vi "Machine Setting - Read Write Machine (SubVI).vi"() -> ()   [LabVIEW 2019]
uses:
  Controls/MachineSetting-state.ctl
  Controls/UDP - Command.ctl
  Controls/Communication - Write Data.ctl
  <vilib>/Utility/sysdir.llb/System Directory Type.ctl
  Controls/Global - Data UDP.vi
  <vilib>/Utility/config.llb/Write Key (String).vi
  <vilib>/Utility/config.llb/Read Key (String).vi
  <vilib>/Utility/config.llb/NI_LVConfig.lvlib
panel:
  in  "Save":bool
  in  "Load":bool
  in  "IP Address":string
  in  "Set":bool
  in  "Get":bool
  in  "Tab Control":enum32{"System", "Test", "ADC", "Sensor", "PID"}(tab)
  in  "System":string[][](table)=[["Out_Type"], ["Inverse"], ["Monitor"], ["ACC_Time"], ["Pulse_rev"], ["Stroke"], ["Auto Off"], ["Gear_Ratio"], ["Pitch"], ["Max Speed"], ["Jog Speed"], ["Disp Coff"], ["Max Load"]]
  in  "Test":string[][](table)=[["Traget #1"], ["Target #2"], ["Speed #1"], ["Speed #2"], [""], [""], [""], [""], [""], [""], [""], [""]]
  in  "ADC":string[][](table)=[["ActiveCH #0"], ["ActiveCH #1"], ["ActiveCH #2"], ["ActiveCH #3"], ["ActiveCH #4"], ["ActiveCH #5"], ["ActiveCH #6"], ["ActiveCH #7"], ["FilterType"], ["PostFilter #0"], ["PostFilter #1"], ["PostFilter #2"], ["PostFilter #3"], ["PostFilter #4"], ["PostFilter #5"], ["PostFilter #6"], ["PostFilter #7"], ["Gain #0"], ["Gain #1"], ["Gain #2"], ["Gain #3"], ["Gain #4"], ["Gain #5"], ["Gain #6"], ["Gain #7"], ["FS"], ["IntOC"], ["IntFC"], ["SysOC"], ["Cofficient #0"], ["Cofficient #1"], ["Cofficient #2"], ["Cofficient #3"], ["Cofficient #4"], ["Cofficient #5"], ["Cofficient #6"], ["Cofficient #7"], ["K1"], ["K2"], ["Max"]]
  in  "Sensor":string[][](table)=[["#1", ""], ["Name", ""], ["SUnit", ""], ["DecPoint", ""], ["Log", ""], ["H_Alarm", ""], ["L_Alarm", ""], ["H_Limit", ""], ["L_Limit", ""], ["Filter", ""], ["Gain", ""], ["Cal Type", " "], ["", ""], ["#2", ""], ["Name", ""], ["SUnit", ""], ["DecPoint", ""], ["Log", ""], ["H_Alarm", ""], ["L_Alarm", ""], ["H_Limit", ""], ["L_Limit", ""], ["Filter", ""], ["Gain", ""], ["Cal Type", ""], ["", ""], ["#3", ""], ["Name", ""], ["SUnit", ""], ["DecPoint", ""], ["Log", ""], ["H_Alarm", ""], ["L_Alarm", ""], ["H_Limit", ""], ["L_Limit", ""], ["Filter", ""], ["Gain", ""], ["Cal Type", ""], ["", ""], ["#4", ""], ["Name", ""], ["SUnit", ""], ["DecPoint", ""], ["Log", ""], ["H_Alarm", ""], ["L_Alarm", ""], ["H_Limit", ""], ["L_Limit", ""], ["Filter", ""], ["Gain", ""], ["Cal Type", ""]]
  in  "PID":string[][](table)=[["SP"], ["PV"], ["KP"], ["KI"], ["KD"], ["FF"], ["Err_Band"], ["Max"], ["Min"], ["Ts"], ["Out"], ["Mode"]]
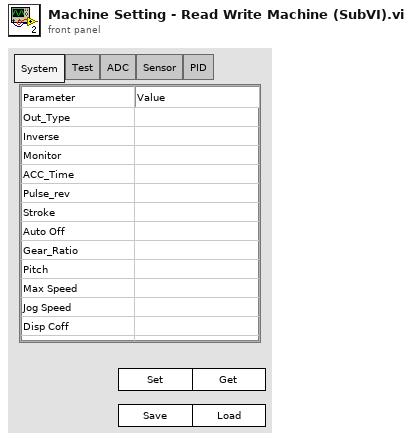
[diagram p1: front panel]
types:
  T1 = typedef "MachineSetting-state.ctl" = enum16{"Init", "Idle", "Get System", "Get Test", "Get ADC", "Get Sensor", "Get PID", "Set System", "Set Test", "Set ADC", "Set Sensor", "Set PID", "Save", "Load", "Exit"}
  T2 = typedef "UDP - Command.ctl" = enum16{"Stop", "Jog Up", "Jog Down", "Ramp Up", "Ramp Down", "PID Target", "PID Ramp", "Disp Run", "Read Ch Data", "Zero Channel", "Zero Disp", "Read Sensor", "Write Sensor", "Read ADC", "Write ADC", "Read PID", "Write PID", "Read Test", "Write Test", "Read System", "Write System", "Read Datalog", "Read Datalog Sensor"}
  T3 = typedef "Communication - Write Data.ctl" = cluster{"Test":cluster{"Target Load":sgl, "Target Disp":sgl, "Rate":sgl, "Speed":sgl}, "Sensor":cluster{"Name":string[], "Unit":string[], "Decimal Point":u8[], "Ch Log":u8[], "H Alarm":u8[], "L Alarm":u8[], "H Limit":sgl[], "L Limit":sgl[], "Filter":u8[], "Gain":u8[], "Calib Type":u32[]}, "PID":cluster{"SP":sgl, "PV":sgl, "kP":sgl, "kI":sgl, "kD":sgl, "FF":sgl, "Err Band":sgl, "Max":i32, "Min":i32, "Ts":u32, "Out":i32, "Mode":u8}, "ADC":cluster{"Active Ch":u8[], "Filter Type":u8, "Post Filter":u8[], "Gain":u8[], "FS":u16, "IntOC":u8, "IntFC":u8, "SysOC":u8, "Cofficient":dbl[], "K":dbl[], "Max":i32}, "System":cluster{"Out Type":u8, "Inverse":u8, "Monitor":u8, "Reserve":u8, "ACC Time":u32, "Pulse Rev":u32, "Stroke":u32, "Auto Off":u32, "Gear Ratio":sgl, "Pitch":sgl, "Max Speed":u32, "Jog Speed":u32, "Disp Coff":sgl, "Max Load":u32}, "Index":enum16{"Ch1", "Ch2", "Ch3", "Ch4", "Ch5", "Ch6", "Ch7", "Ch8", "Ch9", "Ch10", "Ch11", "Ch12", "Ch13", "Ch14", "Ch15", "Ch16"}, "Datalog":enum16{"Ch1-Ch16", "Ch17-Ch32", "Ch32-Ch48", "Ch49-Ch64", "Empty"}}
  T4 = cluster{"Out Type":u8, "Inverse":u8, "Monitor":u8, "Reserve":u8, "ACC Time":u32, "Pulse Rev":u32, "Stroke":u32, "Auto Off":u32, "Gear Ratio":sgl, "Pitch":sgl, "Max Speed":u32, "Jog Speed":u32, "Disp Coff":sgl, "Max Load":u32}
  T5 = cluster{"Target Load":sgl, "Target Disp":sgl, "Rate":sgl, "Speed":sgl}
  T6 = cluster{"Active Ch":u8[], "Filter Type":u8, "Post Filter":u8[], "Gain":u8[], "FS":u16, "IntOC":u8, "IntFC":u8, "SysOC":u8, "Cofficient":dbl[], "K":dbl[], "Max":i32}
  T7 = cluster{"Name":string[], "Unit":string[], "Decimal Point":u8[], "Ch Log":u8[], "H Alarm":u8[], "L Alarm":u8[], "H Limit":sgl[], "L Limit":sgl[], "Filter":u8[], "Gain":u8[], "Calib Type":u32[]}
  T8 = cluster{"SP":sgl, "PV":sgl, "kP":sgl, "kI":sgl, "kD":sgl, "FF":sgl, "Err Band":sgl, "Max":i32, "Min":i32, "Ts":u32, "Out":i32, "Mode":u8}
  T9 = cluster{"Out Type":string, "Inverse":string, "Monitor":string, "Reserve":string, "ACC Time":string, "Pulse Rev":string, "Stroke":string, "Auto Off":string, "Gear Ratio":string, "Pitch":string, "Max Speed":string, "Jog Speed":string, "Disp Coff":string, "Max Load":string}
  T10 = cluster{"Target Load":string, "Target Disp":string, "Rate":string, "Speed":string}
  T11 = cluster{"SP":string, "PV":string, "kP":string, "kI":string, "kD":string, "FF":string, "Err Band":string, "Max":string, "Min":string, "Ts":string, "Out":string, "Mode":string}
  T12 = typedef "System Directory Type.ctl" = i32
  T13 = typedef "NI_LVConfig.lvlib/Config Data RefNum.ctl" = refnum<k1>
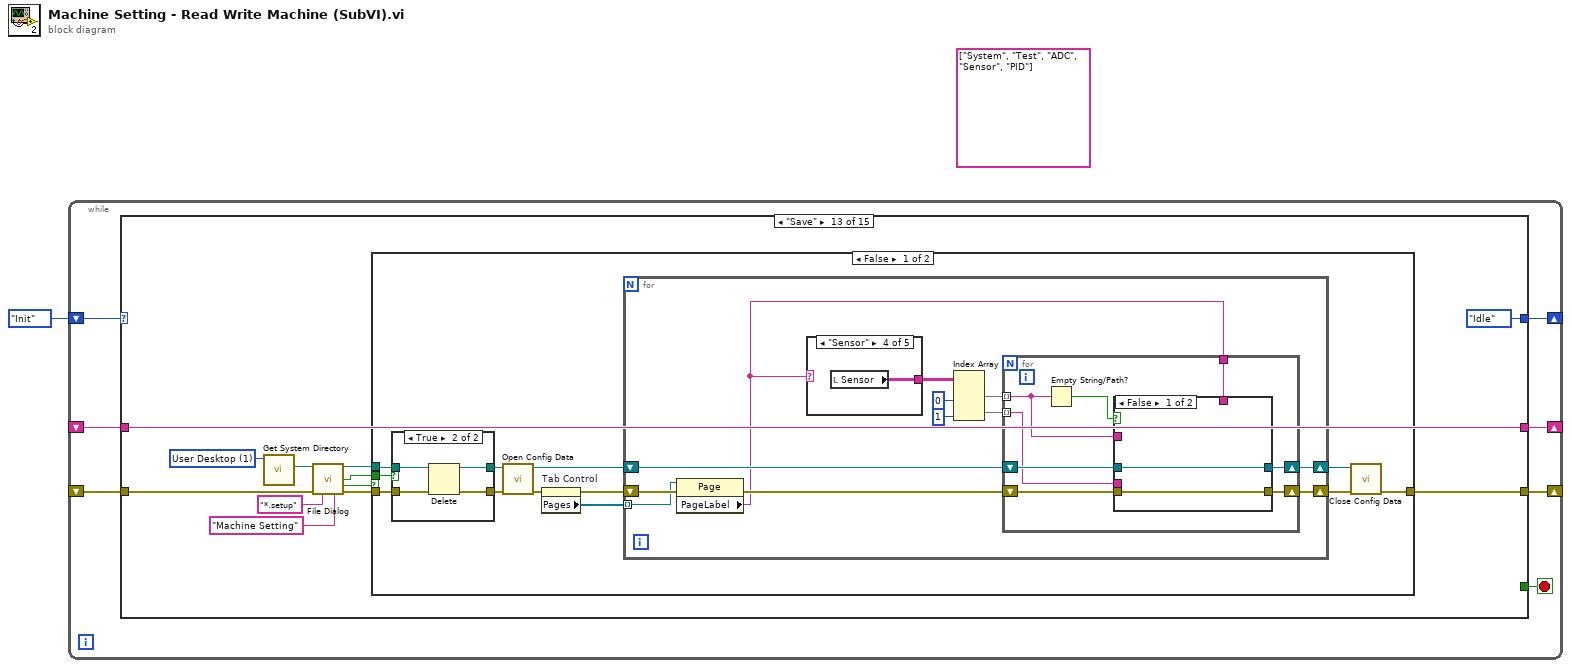
[diagram p0: block diagram]
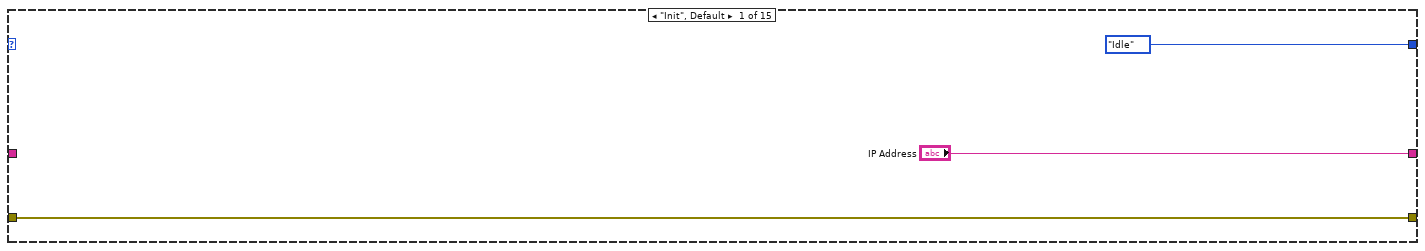
[diagram p2: hidden frame]
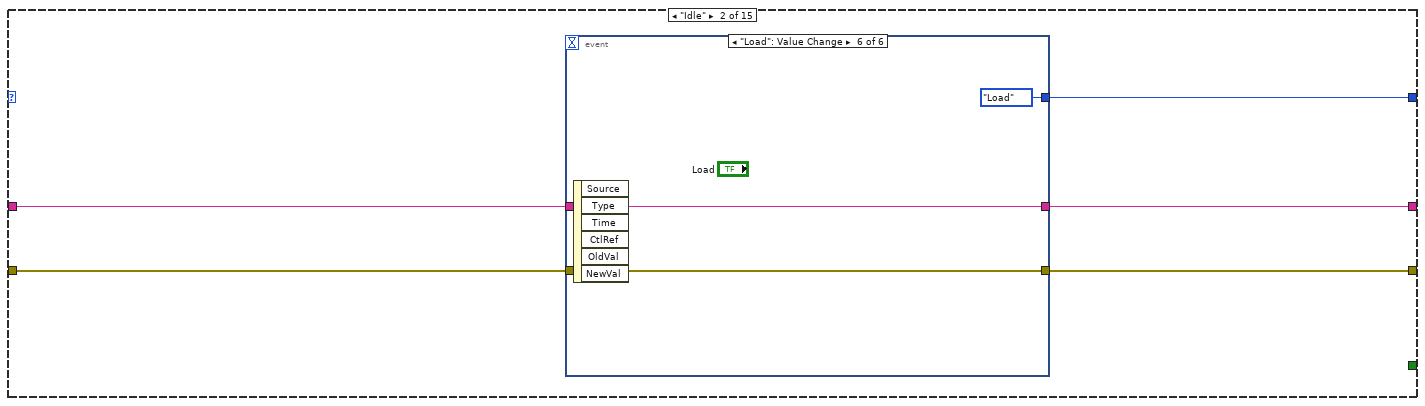
[diagram p3: hidden frame]
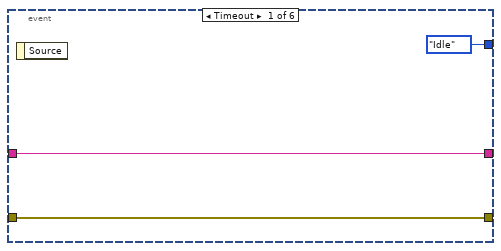
[diagram p4: hidden frame]
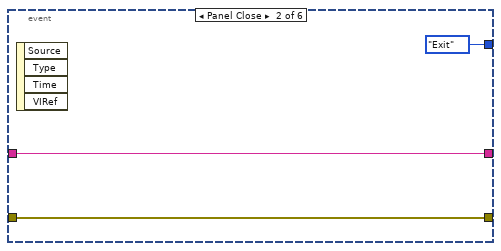
[diagram p5: hidden frame]
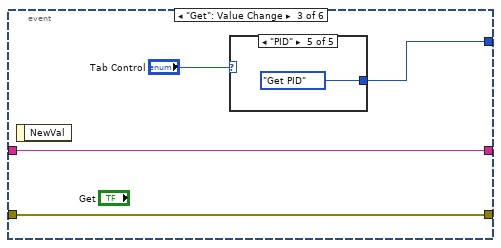
[diagram p6: hidden frame]
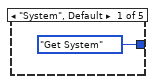
[diagram p7: hidden frame]
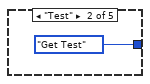
[diagram p8: hidden frame]
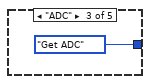
[diagram p9: hidden frame]
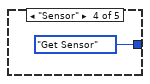
[diagram p10: hidden frame]
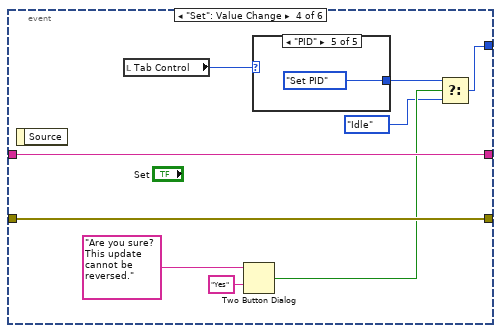
[diagram p11: hidden frame]
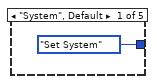
[diagram p12: hidden frame]
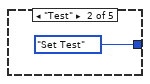
[diagram p13: hidden frame]
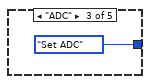
[diagram p14: hidden frame]
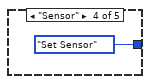
[diagram p15: hidden frame]
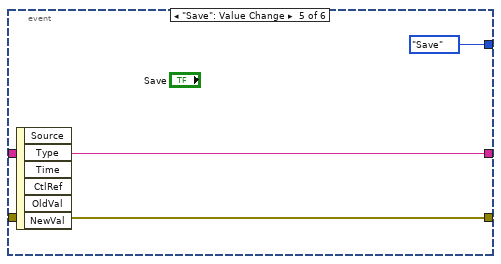
[diagram p16: hidden frame]
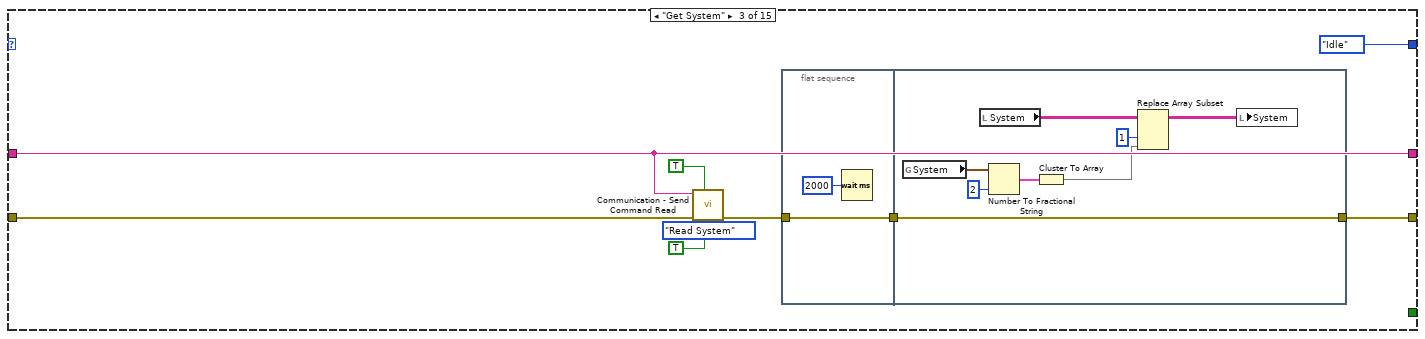
[diagram p17: hidden frame]
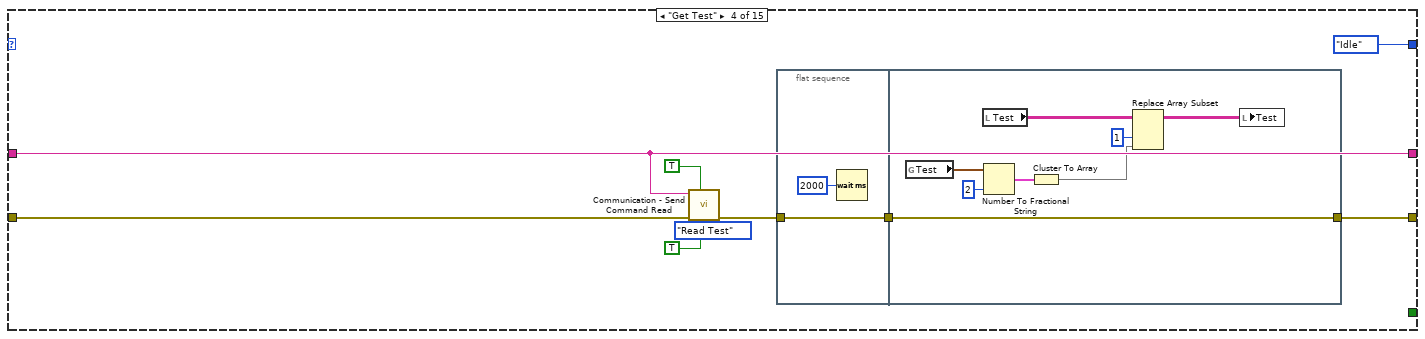
[diagram p18: hidden frame]
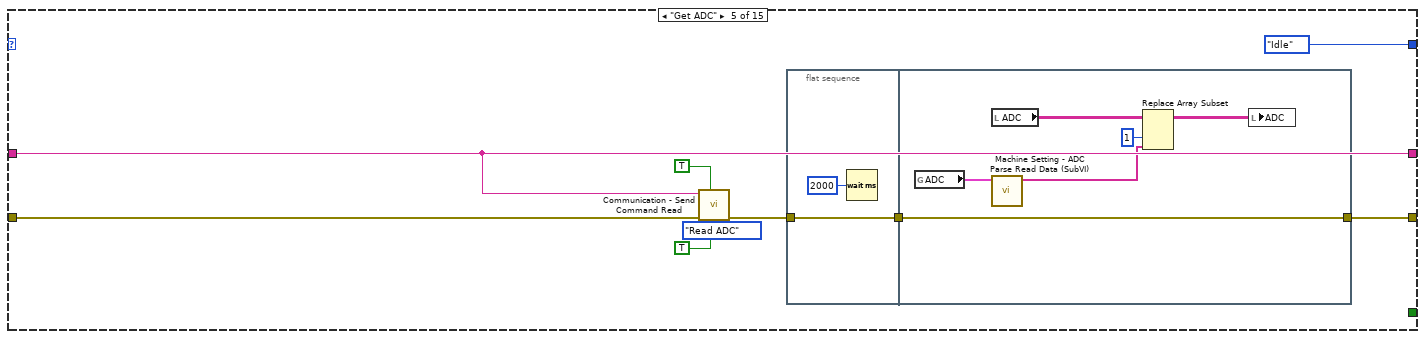
[diagram p19: hidden frame]
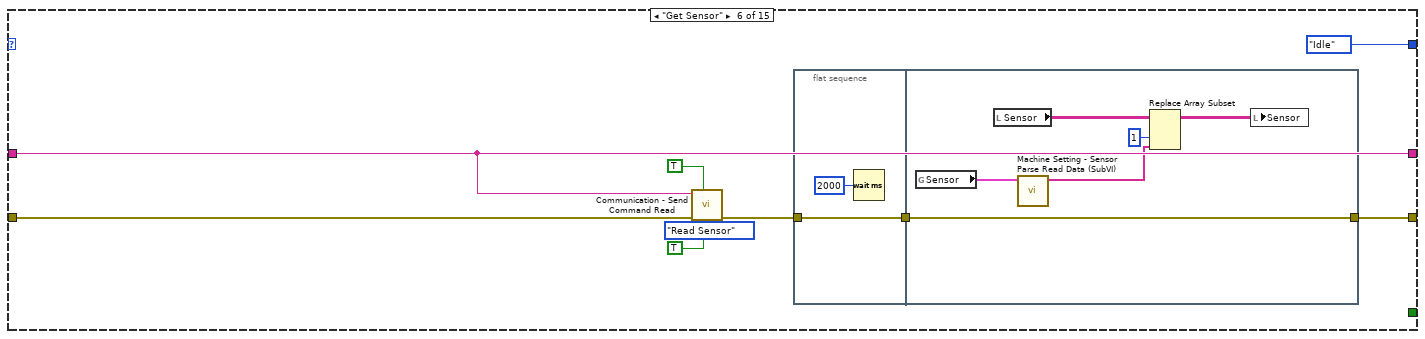
[diagram p20: hidden frame]
diagram:
  (unwired) string[] ["System", "Test", "ADC", "Sensor", "PID"] ("Array")
  n1 = while {
    shift-right: [w7] -> _
    shift-left: _ -> [w6]
    shift-right: [w5] -> _
    shift-left: _ -> [w4]
    shift-right: [w2] -> _
    shift-left: MachineSetting-state."Init" ("f") -> [w3]
    stop <- w8 stop-if-true
    n2 = case shown="\"Save\"" w3 {
      tunnel: [MachineSetting-state."Idle" ("f") w16 MachineSetting-state."Idle" ("f") MachineSetting-state."Idle" ("f") MachineSetting-state."Idle" ("f") MachineSetting-state."Idle" ("f") MachineSetting-state."Idle" ("f") MachineSetting-state."Idle" ("f") MachineSetting-state."Idle" ("f") MachineSetting-state."Idle" ("f") MachineSetting-state."Idle" ("f") MachineSetting-state."Idle" ("f") MachineSetting-state."Idle" ("f") MachineSetting-state."Idle" ("f") MachineSetting-state."Exit" ("f")] -> w2
      tunnel: [_ _ _ _ _ _ _ _ _ _ _ _ _ _ TRUE] -> w8
      tunnel: ["IP Address" w14 w58 w75 w94 w111 w128 w151 w234 w272 w594 w691 w772 w830 "" ("IP Address")] -> w7
      tunnel: w6 -> [_ w15 w58 w75 w94 w111 w128 w151 w234 w272 w594 w691 w772 w830 _]
      tunnel: [w10 w13 w55 w72 w91 w108 w125 w152 w235 w273 w599 w692 w765 w829 w887] -> w5
      tunnel: w4 -> [w10 w12 w59 w76 w95 w112 w129 w153 w236 w274 w593 w693 w770 w836 w887]
      frame "Init", Default {
      }
      frame "Idle" {
        n3 = event shown="[5] \"Load\": Value Change" {
          selector: _ -> [_ _ _ _ _ _]
          dyn-events: _ -> [_ _ _ _ _ _]
          timeout: _ -> [_ _ _ _ _ _]
          tunnel: [MachineSetting-state."Idle" ("f") MachineSetting-state."Exit" ("f") w25 w33 MachineSetting-state."Save" ("f") MachineSetting-state."Load" ("f")] -> w16
          tunnel: w15 -> [w19 w22 w24 w39 w48 w51]
          tunnel: [w19 w22 w24 w39 w48 w51] -> w14
          tunnel: [w18 w21 w23 w38 w47 w50] -> w13
          tunnel: w12 -> [w18 w21 w23 w38 w47 w50]
          event Timeout {
            n4 = event-data() -> ()  [unwired: 1 in, 1 out]
          }
          event Panel Close {
            n5 = event-data() -> ()  [unwired: 1 in, 4 out]
          }
          event "Get": Value Change {
            n6 = event-data() -> ()  [unwired: 1 in, 1 out]
            n7 = case shown="\"PID\"" "Tab Control" {
              tunnel: [MachineSetting-state."Get System" MachineSetting-state."Get Test" MachineSetting-state."Get ADC" MachineSetting-state."Get Sensor" MachineSetting-state."Get PID"] -> w25
              frame "System", Default {
              }
              frame "Test" {
              }
              frame "ADC" {
              }
              frame "Sensor" {
              }
              frame "PID" {
              }
            }
          }
          event "Set": Value Change {
            n8 = event-data() -> ()  [unwired: 1 in, 1 out]
            n9 = local read "Tab Control"() -> (w40:enum32{"System", "Test", "ADC", "Sensor", "PID"})
            n10 = Two Button Dialog(message="Are you sure? This update cannot be reversed.", 2:"Yes" ("T button name (\"OK\")")) -> (T button?=w35:bool)  [unwired: 1 in]
            n11 = case shown="\"PID\"" w40 {
              tunnel: [MachineSetting-state."Set System" MachineSetting-state."Set Test" MachineSetting-state."Set ADC" MachineSetting-state."Set Sensor" MachineSetting-state."Set PID"] -> w34
              frame "System", Default {
              }
              frame "Test" {
              }
              frame "ADC" {
              }
              frame "Sensor" {
              }
              frame "PID" {
              }
            }
            n12 = Select(t=w34, s=w35, f=MachineSetting-state."Idle") -> (s? t:f=w33:T1)
          }
          event "Save": Value Change {
            n13 = event-data() -> ()  [unwired: 1 in, 6 out]
          }
          event "Load": Value Change {
            n14 = event-data() -> ()  [unwired: 1 in, 6 out]
          }
        }
      }
      frame "Get System" {
        n15 = call "Communication - Send Command Read.vi"("Fron?"=TRUE, "Bypass?"=TRUE, "error in (no error)"=w59, "Action"=UDP_-_Command."Read System", "Device IP Address"=w58) -> ("error out"=w53:errorcluster)  [unwired: 6 in]
        n16 = flat-sequence {
          tunnel: [w61] -> w54
          tunnel: w53 -> [w61]
          tunnel: [w63] -> w55
          tunnel: w54 -> [w63]
          frame #0 {
            n17 = Wait (ms)(milliseconds to wait=u32 2000) -> ()  [unwired: 1 out]
          }
          frame #1 {
            n18 = global read "Global - Data UDP.vi" "System"() -> (w67:T4)
            n19 = local read "System"() -> (w70:string[][])
            n20 = Number To Fractional String(number=w67, precision (6)=i16 2) -> (F-format string=w65:T9)  [unwired: 2 in]
            n21 = Cluster To Array(cluster=w65) -> (array=w64:string[])
            n22 = Replace Array Subset(array=w70, new element=w64, index (col)=1 ("disabled index (col)")) -> (w69:string[][])  [unwired: 1 in]
            n23 = local write "System"(w69) -> ()
          }
        }
      }
      frame "Get Test" {
        n24 = call "Communication - Send Command Read.vi"("Fron?"=TRUE, "Bypass?"=TRUE, "error in (no error)"=w76, "Action"=UDP_-_Command."Read Test", "Device IP Address"=w75) -> ("error out"=w73:errorcluster)  [unwired: 6 in]
        n25 = flat-sequence {
          tunnel: [w80] -> w74
          tunnel: w73 -> [w80]
          tunnel: [w82] -> w72
          tunnel: w74 -> [w82]
          frame #0 {
            n26 = Wait (ms)(milliseconds to wait=u32 2000) -> ()  [unwired: 1 out]
          }
          frame #1 {
            n27 = global read "Global - Data UDP.vi" "Test"() -> (w86:T5)
            n28 = local read "Test"() -> (w89:string[][])
            n29 = Number To Fractional String(number=w86, precision (6)=i16 2) -> (F-format string=w84:T10)  [unwired: 2 in]
            n30 = Cluster To Array(cluster=w84) -> (array=w83:string[])
            n31 = Replace Array Subset(array=w89, new element=w83, index (col)=1 ("disabled index (col)")) -> (w88:string[][])  [unwired: 1 in]
            n32 = local write "Test"(w88) -> ()
          }
        }
      }
      frame "Get ADC" {
        n33 = call "Communication - Send Command Read.vi"("Fron?"=TRUE, "Bypass?"=TRUE, "error in (no error)"=w95, "Action"=UDP_-_Command."Read ADC", "Device IP Address"=w94) -> ("error out"=w92:errorcluster)  [unwired: 6 in]
        n34 = flat-sequence {
          tunnel: [w99] -> w93
          tunnel: w92 -> [w99]
          tunnel: [w103] -> w91
          tunnel: w93 -> [w103]
          frame #0 {
            n35 = Wait (ms)(milliseconds to wait=u32 2000) -> ()  [unwired: 1 out]
          }
          frame #1 {
            n36 = global read "Global - Data UDP.vi" "ADC"() -> (w102:T6)
            n37 = local read "ADC"() -> (w106:string[][])
            n38 = call "Machine Setting - ADC Parse Read Data (SubVI).vi"("ADC"=w102) -> ("Array"=w101:string[])  [unwired: 10 in]
            n39 = Replace Array Subset(array=w106, new element=w101, index (col)=1 ("disabled index (col)")) -> (w105:string[][])  [unwired: 1 in]
            n40 = local write "ADC"(w105) -> ()
          }
        }
      }
      frame "Get Sensor" {
        n41 = call "Communication - Send Command Read.vi"("Fron?"=TRUE, "Bypass?"=TRUE, "error in (no error)"=w112, "Action"=UDP_-_Command."Read Sensor", "Device IP Address"=w111) -> ("error out"=w109:errorcluster)  [unwired: 6 in]
        n42 = flat-sequence {
          tunnel: [w116] -> w110
          tunnel: w109 -> [w116]
          tunnel: [w120] -> w108
          tunnel: w110 -> [w120]
          frame #0 {
            n43 = Wait (ms)(milliseconds to wait=u32 2000) -> ()  [unwired: 1 out]
          }
          frame #1 {
            n44 = global read "Global - Data UDP.vi" "Sensor"() -> (w119:T7)
            n45 = local read "Sensor"() -> (w123:string[][])
            n46 = call "Machine Setting - Sensor Parse Read Data (SubVI).vi"("Sensor"=w119) -> ("Array"=w118:string[])  [unwired: 10 in]
            n47 = Replace Array Subset(array=w123, new element=w118, index (col)=1 ("disabled index (col)")) -> (w122:string[][])  [unwired: 1 in]
            n48 = local write "Sensor"(w122) -> ()
          }
        }
      }
      frame "Get PID" {
        n49 = call "Communication - Send Command Read.vi"("Fron?"=TRUE, "Bypass?"=TRUE, "error in (no error)"=w129, "Action"=UDP_-_Command."Read PID", "Device IP Address"=w128) -> ("error out"=w126:errorcluster)  [unwired: 6 in]
        n50 = flat-sequence {
          tunnel: [w133] -> w127
          tunnel: w126 -> [w133]
          tunnel: [w135] -> w125
          tunnel: w127 -> [w135]
          frame #0 {
            n51 = Wait (ms)(milliseconds to wait=u32 2000) -> ()  [unwired: 1 out]
          }
          frame #1 {
            n52 = global read "Global - Data UDP.vi" "PID"() -> (w139:T8)
            n53 = Number To Fractional String(number=w139, precision (6)=i16 2) -> (F-format string=w137:T11)  [unwired: 2 in]
            n54 = local read "PID"() -> (w142:string[][])
            n55 = Cluster To Array(cluster=w137) -> (array=w136:string[])
            n56 = Replace Array Subset(array=w142, new element=w136, index (col)=1 ("disabled index (col)")) -> (w141:string[][])  [unwired: 1 in]
            n57 = local write "PID"(w141) -> ()
          }
        }
      }
      frame "Set System" {
        n58 = Index Array(array="System", index (col)=1 ("disabled index (col)")) -> (element=w148:string[])  [unwired: 1 in]
        n59 = for {
          tunnel: w148 -> [w159] mode=indexing
          shift-right: [w157] -> w146
          shift-left: T4 {"Out Type"=0, "Inverse"=0, "Monitor"=0, "Reserve"=0, "ACC Time"=0, "Pulse Rev"=0, "Stroke"=0, "Auto Off"=0, "Gear Ratio"=0.0, "Pitch"=0.0, "Max Speed"=0, "Jog Speed"=0, "Disp Coff"=0.0, "Max Load"=0} ("System") -> [w158]
          i -> [w160]
          n60 = case shown="4" w160 {
            tunnel: w159 -> [w164 w169 w174 w180 w185 w190 w195 w200 w205 w210 w215 w220 w225]
            tunnel: w158 -> [w163 w168 w173 w179 w184 w189 w194 w199 w204 w209 w214 w219 w224]
            tunnel: [w161 w166 w171 w178 w182 w187 w192 w197 w202 w207 w212 w217 w222] -> w157
            frame 0, Default {
              n61 = Decimal String To Number(string=w164, default (0L)=u8 0 ("Out Type")) -> (number=w162:u8)  [unwired: 1 in, 1 out]
              n62 = Bundle By Name(cluster=w163, "Out Type"=w162) -> (w161:T4)
            }
            frame 1 {
              n63 = Decimal String To Number(string=w169, default (0L)=u8 0 ("Out Type")) -> (number=w167:u8)  [unwired: 1 in, 1 out]
              n64 = Bundle By Name(cluster=w168, "Inverse"=w167) -> (w166:T4)
            }
            frame 2 {
              n65 = Decimal String To Number(string=w174, default (0L)=u8 0 ("Out Type")) -> (number=w172:u8)  [unwired: 1 in, 1 out]
              n66 = Bundle By Name(cluster=w173, "Monitor"=w172) -> (w171:T4)
            }
            frame 3 {
              n67 = Decimal String To Number(string=w180, default (0L)=u32 0 ("ACC Time")) -> (number=w176:u32)  [unwired: 1 in, 1 out]
              n68 = Bundle By Name(cluster=w179, "ACC Time"=w176) -> (w178:T4)
            }
            frame 4 {
              n69 = Decimal String To Number(string=w185, default (0L)=u32 0 ("ACC Time")) -> (number=w183:u32)  [unwired: 1 in, 1 out]
              n70 = Bundle By Name(cluster=w184, "Pulse Rev"=w183) -> (w182:T4)
            }
            frame 5 {
              n71 = Decimal String To Number(string=w190, default (0L)=u32 0 ("ACC Time")) -> (number=w188:u32)  [unwired: 1 in, 1 out]
              n72 = Bundle By Name(cluster=w189, "Stroke"=w188) -> (w187:T4)
            }
            frame 6 {
              n73 = Decimal String To Number(string=w195, default (0L)=u32 0 ("ACC Time")) -> (number=w193:u32)  [unwired: 1 in, 1 out]
              n74 = Bundle By Name(cluster=w194, "Auto Off"=w193) -> (w192:T4)
            }
            frame 7 {
              n75 = Fract/Exp String To Number(string=w200, default (0 dbl)=sgl 0.0 ("ACC Time")) -> (number=w198:sgl)  [unwired: 2 in, 1 out]
              n76 = Bundle By Name(cluster=w199, "Gear Ratio"=w198) -> (w197:T4)
            }
            frame 8 {
              n77 = Fract/Exp String To Number(string=w205, default (0 dbl)=sgl 0.0 ("ACC Time")) -> (number=w203:sgl)  [unwired: 2 in, 1 out]
              n78 = Bundle By Name(cluster=w204, "Pitch"=w203) -> (w202:T4)
            }
            frame 9 {
              n79 = Decimal String To Number(string=w210, default (0L)=u32 0 ("ACC Time")) -> (number=w208:u32)  [unwired: 1 in, 1 out]
              n80 = Bundle By Name(cluster=w209, "Max Speed"=w208) -> (w207:T4)
            }
            frame 10 {
              n81 = Decimal String To Number(string=w215, default (0L)=u32 0 ("ACC Time")) -> (number=w213:u32)  [unwired: 1 in, 1 out]
              n82 = Bundle By Name(cluster=w214, "Jog Speed"=w213) -> (w212:T4)
            }
            frame 11 {
              n83 = Fract/Exp String To Number(string=w220, default (0 dbl)=sgl 0.0 ("ACC Time")) -> (number=w218:sgl)  [unwired: 2 in, 1 out]
              n84 = Bundle By Name(cluster=w219, "Disp Coff"=w218) -> (w217:T4)
            }
            frame 12 {
              n85 = Decimal String To Number(string=w225, default (0L)=u32 0 ("ACC Time")) -> (number=w223:u32)  [unwired: 1 in, 1 out]
              n86 = Bundle By Name(cluster=w224, "Max Load"=w223) -> (w222:T4)
            }
          }
        }
        n87 = Bundle By Name(cluster=T3 {"Test"={"Target Load"=0.0, "Target Disp"=0.0, "Rate"=0.0, "Speed"=0.0}, "Sensor"={"Name"=[], "Unit"=[], "Decimal Point"=[], "Ch Log"=[], "H Alarm"=[], "L Alarm"=[], "H Limit"=[], "L Limit"=[], "Filter"=[], "Gain"=[], "Calib Type"=[]}, "PID"={"SP"=0.0, "PV"=0.0, "kP"=0.0, "kI"=0.0, "kD"=0.0, "FF"=0.0, "Err Band"=0.0, "Max"=0, "Min"=0, "Ts"=0, "Out"=0, "Mode"=0}, "ADC"={"Active Ch"=[], "Filter Type"=0, "Post Filter"=[], "Gain"=[], "FS"=0, "IntOC"=0, "IntFC"=0, "SysOC"=0, "Cofficient"=[], "K"=[], "Max"=0}, "System"={"Out Type"=0, "Inverse"=0, "Monitor"=0, "Reserve"=0, "ACC Time"=0, "Pulse Rev"=0, "Stroke"=0, "Auto Off"=0, "Gear Ratio"=0.0, "Pitch"=0.0, "Max Speed"=0, "Jog Speed"=0, "Disp Coff"=0.0, "Max Load"=0}, "Index"=enum."Ch1", "Datalog"=enum."Empty"} ("Data"), "System"=w146) -> (w144:T3)
        n88 = call "Communication - Send Command Read.vi"("Fron?"=TRUE, "Bypass?"=TRUE, "error in (no error)"=w153, "Data"=w144, "Action"=UDP_-_Command."Write System", "Device IP Address"=w151) -> ("error out"=w152:errorcluster)  [unwired: 5 in]
      }
      frame "Set Test" {
        n89 = Index Array(array="Test", index (col)=1 ("disabled index (col)")) -> (element=w231:string[])  [unwired: 1 in]
        n90 = for {
          tunnel: w231 -> [w242] mode=indexing
          shift-right: [w240] -> w228
          shift-left: T5 {"Target Load"=0.0, "Target Disp"=0.0, "Rate"=0.0, "Speed"=0.0} ("Test") -> [w241]
          i -> [w243]
          n91 = case shown="3" w243 {
            tunnel: w242 -> [w246 w251 w256 w261]
            tunnel: w241 -> [w248 w253 w258 w263]
            tunnel: [w247 w252 w257 w262] -> w240
            frame 0, Default {
              n92 = Fract/Exp String To Number(string=w246, default (0 dbl)=sgl 0.0 ("default (0 DBL)")) -> (number=w245:sgl)  [unwired: 2 in, 1 out]
              n93 = Bundle By Name(cluster=w248, "Target Load"=w245) -> (w247:T5)
            }
            frame 1 {
              n94 = Fract/Exp String To Number(string=w251, default (0 dbl)=sgl 0.0 ("default (0 DBL)")) -> (number=w250:sgl)  [unwired: 2 in, 1 out]
              n95 = Bundle By Name(cluster=w253, "Target Disp"=w250) -> (w252:T5)
            }
            frame 2 {
              n96 = Fract/Exp String To Number(string=w256, default (0 dbl)=sgl 0.0 ("default (0 DBL)")) -> (number=w255:sgl)  [unwired: 2 in, 1 out]
              n97 = Bundle By Name(cluster=w258, "Rate"=w255) -> (w257:T5)
            }
            frame 3 {
              n98 = Fract/Exp String To Number(string=w261, default (0 dbl)=sgl 0.0 ("default (0 DBL)")) -> (number=w260:sgl)  [unwired: 2 in, 1 out]
              n99 = Bundle By Name(cluster=w263, "Speed"=w260) -> (w262:T5)
            }
          }
        }
        n100 = Bundle By Name(cluster=T3 {"Test"={"Target Load"=0.0, "Target Disp"=0.0, "Rate"=0.0, "Speed"=0.0}, "Sensor"={"Name"=[], "Unit"=[], "Decimal Point"=[], "Ch Log"=[], "H Alarm"=[], "L Alarm"=[], "H Limit"=[], "L Limit"=[], "Filter"=[], "Gain"=[], "Calib Type"=[]}, "PID"={"SP"=0.0, "PV"=0.0, "kP"=0.0, "kI"=0.0, "kD"=0.0, "FF"=0.0, "Err Band"=0.0, "Max"=0, "Min"=0, "Ts"=0, "Out"=0, "Mode"=0}, "ADC"={"Active Ch"=[], "Filter Type"=0, "Post Filter"=[], "Gain"=[], "FS"=0, "IntOC"=0, "IntFC"=0, "SysOC"=0, "Cofficient"=[], "K"=[], "Max"=0}, "System"={"Out Type"=0, "Inverse"=0, "Monitor"=0, "Reserve"=0, "ACC Time"=0, "Pulse Rev"=0, "Stroke"=0, "Auto Off"=0, "Gear Ratio"=0.0, "Pitch"=0.0, "Max Speed"=0, "Jog Speed"=0, "Disp Coff"=0.0, "Max Load"=0}, "Index"=enum."Ch1", "Datalog"=enum."Empty"} ("Data"), "Test"=w228) -> (w227:T3)
        n101 = call "Communication - Send Command Read.vi"("Fron?"=TRUE, "Bypass?"=TRUE, "error in (no error)"=w236, "Data"=w227, "Action"=UDP_-_Command."Write Test", "Device IP Address"=w234) -> ("error out"=w235:errorcluster)  [unwired: 5 in]
      }
      frame "Set ADC" {
        n102 = Index Array(array="ADC", index (col)=1 ("disabled index (col)")) -> (element=w270:string[])  [unwired: 1 in]
        n103 = for {
          tunnel: w270 -> [w280] mode=indexing
          shift-right: [w278] -> w268
          shift-left: T6 {"Active Ch"=[0, 0, 0, 0, 0, 0, 0, 0], "Filter Type"=0, "Post Filter"=[0, 0, 0, 0, 0, 0, 0, 0], "Gain"=[0, 0, 0, 0, 0, 0, 0, 0], "FS"=0, "IntOC"=0, "IntFC"=0, "SysOC"=0, "Cofficient"=[0.0, 0.0, 0.0, 0.0, 0.0, 0.0, 0.0, 0.0], "K"=[0.0, 0.0, 0.0, 0.0, 0.0, 0.0, 0.0, 0.0], "Max"=0} ("ADC") -> [w279]
          i -> [w281]
          n104 = case shown="3" w281 {
            tunnel: w280 -> [w288 w296 w304 w312 w320 w328 w336 w344 w349 w357 w365 w373 w381 w389 w397 w405 w413 w421 w429 w437 w445 w453 w461 w469 w477 w482 w487 w492 w497 w505 w513 w521 w529 w537 w545 w553 w561 w569 w577 w582]
            tunnel: w279 -> [w286 w294 w302 w310 w318 w326 w334 w342 w347 w355 w363 w371 w379 w387 w395 w403 w411 w419 w427 w435 w443 w451 w459 w467 w475 w480 w485 w490 w495 w503 w511 w519 w527 w535 w543 w551 w559 w567 w575 w581]
            tunnel: [w289 w297 w305 w313 w321 w329 w337 w345 w350 w358 w366 w374 w382 w390 w398 w406 w414 w422 w430 w438 w446 w454 w462 w470 w478 w483 w488 w493 w498 w506 w514 w522 w530 w538 w546 w554 w562 w570 w578 w583] -> w278
            frame 0, Default {
              n105 = Unbundle By Name(w286) -> ("Active Ch"=w285:u8[])
              n106 = Decimal String To Number(string=w288, default (0L)=u8 0 ("default (0 DBL)")) -> (number=w282:u8)  [unwired: 1 in, 1 out]
              n107 = Replace Array Subset(array=w285, new element=w282, index=0) -> (w284:u8[])
              n108 = Bundle By Name(cluster=w286, "Active Ch"=w284) -> (w289:T6)
            }
            frame 1 {
              n109 = Unbundle By Name(w294) -> ("Active Ch"=w293:u8[])
              n110 = Decimal String To Number(string=w296, default (0L)=u8 0 ("default (0 DBL)")) -> (number=w290:u8)  [unwired: 1 in, 1 out]
              n111 = Replace Array Subset(array=w293, new element=w290, index=1) -> (w292:u8[])
              n112 = Bundle By Name(cluster=w294, "Active Ch"=w292) -> (w297:T6)
            }
            frame 2 {
              n113 = Unbundle By Name(w302) -> ("Active Ch"=w301:u8[])
              n114 = Decimal String To Number(string=w304, default (0L)=u8 0 ("default (0 DBL)")) -> (number=w298:u8)  [unwired: 1 in, 1 out]
              n115 = Replace Array Subset(array=w301, new element=w298, index=2) -> (w300:u8[])
              n116 = Bundle By Name(cluster=w302, "Active Ch"=w300) -> (w305:T6)
            }
            frame 3 {
              n117 = Unbundle By Name(w310) -> ("Active Ch"=w309:u8[])
              n118 = Decimal String To Number(string=w312, default (0L)=u8 0 ("default (0 DBL)")) -> (number=w306:u8)  [unwired: 1 in, 1 out]
              n119 = Replace Array Subset(array=w309, new element=w306, index=3) -> (w308:u8[])
              n120 = Bundle By Name(cluster=w310, "Active Ch"=w308) -> (w313:T6)
            }
            frame 4 {
              n121 = Unbundle By Name(w318) -> ("Active Ch"=w317:u8[])
              n122 = Decimal String To Number(string=w320, default (0L)=u8 0 ("default (0 DBL)")) -> (number=w314:u8)  [unwired: 1 in, 1 out]
              n123 = Replace Array Subset(array=w317, new element=w314, index=4) -> (w316:u8[])
              n124 = Bundle By Name(cluster=w318, "Active Ch"=w316) -> (w321:T6)
            }
            frame 5 {
              n125 = Unbundle By Name(w326) -> ("Active Ch"=w325:u8[])
              n126 = Decimal String To Number(string=w328, default (0L)=u8 0 ("default (0 DBL)")) -> (number=w322:u8)  [unwired: 1 in, 1 out]
              n127 = Replace Array Subset(array=w325, new element=w322, index=5) -> (w324:u8[])
              n128 = Bundle By Name(cluster=w326, "Active Ch"=w324) -> (w329:T6)
            }
            frame 6 {
              n129 = Unbundle By Name(w334) -> ("Active Ch"=w333:u8[])
              n130 = Decimal String To Number(string=w336, default (0L)=u8 0 ("default (0 DBL)")) -> (number=w330:u8)  [unwired: 1 in, 1 out]
              n131 = Replace Array Subset(array=w333, new element=w330, index=6) -> (w332:u8[])
              n132 = Bundle By Name(cluster=w334, "Active Ch"=w332) -> (w337:T6)
            }
            frame 7 {
              n133 = Unbundle By Name(w342) -> ("Active Ch"=w341:u8[])
              n134 = Decimal String To Number(string=w344, default (0L)=u8 0 ("default (0 DBL)")) -> (number=w338:u8)  [unwired: 1 in, 1 out]
              n135 = Replace Array Subset(array=w341, new element=w338, index=7) -> (w340:u8[])
              n136 = Bundle By Name(cluster=w342, "Active Ch"=w340) -> (w345:T6)
            }
            frame 8 {
              n137 = Decimal String To Number(string=w349, default (0L)=u8 0 ("default (0 DBL)")) -> (number=w346:u8)  [unwired: 1 in, 1 out]
              n138 = Bundle By Name(cluster=w347, "Filter Type"=w346) -> (w350:T6)
            }
            frame 9 {
              n139 = Unbundle By Name(w355) -> ("Post Filter"=w354:u8[])
              n140 = Decimal String To Number(string=w357, default (0L)=u8 0 ("default (0 DBL)")) -> (number=w351:u8)  [unwired: 1 in, 1 out]
              n141 = Replace Array Subset(array=w354, new element=w351, index=0) -> (w353:u8[])
              n142 = Bundle By Name(cluster=w355, "Post Filter"=w353) -> (w358:T6)
            }
            frame 10 {
              n143 = Unbundle By Name(w363) -> ("Post Filter"=w362:u8[])
              n144 = Decimal String To Number(string=w365, default (0L)=u8 0 ("default (0 DBL)")) -> (number=w359:u8)  [unwired: 1 in, 1 out]
              n145 = Replace Array Subset(array=w362, new element=w359, index=1) -> (w361:u8[])
              n146 = Bundle By Name(cluster=w363, "Post Filter"=w361) -> (w366:T6)
            }
            frame 11 {
              n147 = Unbundle By Name(w371) -> ("Post Filter"=w370:u8[])
              n148 = Decimal String To Number(string=w373, default (0L)=u8 0 ("default (0 DBL)")) -> (number=w367:u8)  [unwired: 1 in, 1 out]
              n149 = Replace Array Subset(array=w370, new element=w367, index=2) -> (w369:u8[])
              n150 = Bundle By Name(cluster=w371, "Post Filter"=w369) -> (w374:T6)
            }
            frame 12 {
              n151 = Unbundle By Name(w379) -> ("Post Filter"=w378:u8[])
              n152 = Decimal String To Number(string=w381, default (0L)=u8 0 ("default (0 DBL)")) -> (number=w375:u8)  [unwired: 1 in, 1 out]
              n153 = Replace Array Subset(array=w378, new element=w375, index=3) -> (w377:u8[])
              n154 = Bundle By Name(cluster=w379, "Post Filter"=w377) -> (w382:T6)
            }
            frame 13 {
              n155 = Unbundle By Name(w387) -> ("Post Filter"=w386:u8[])
              n156 = Decimal String To Number(string=w389, default (0L)=u8 0 ("default (0 DBL)")) -> (number=w383:u8)  [unwired: 1 in, 1 out]
              n157 = Replace Array Subset(array=w386, new element=w383, index=4) -> (w385:u8[])
              n158 = Bundle By Name(cluster=w387, "Post Filter"=w385) -> (w390:T6)
            }
            frame 14 {
              n159 = Unbundle By Name(w395) -> ("Post Filter"=w394:u8[])
              n160 = Decimal String To Number(string=w397, default (0L)=u8 0 ("default (0 DBL)")) -> (number=w391:u8)  [unwired: 1 in, 1 out]
              n161 = Replace Array Subset(array=w394, new element=w391, index=5) -> (w393:u8[])
              n162 = Bundle By Name(cluster=w395, "Post Filter"=w393) -> (w398:T6)
            }
            frame 15 {
              n163 = Unbundle By Name(w403) -> ("Post Filter"=w402:u8[])
              n164 = Decimal String To Number(string=w405, default (0L)=u8 0 ("default (0 DBL)")) -> (number=w399:u8)  [unwired: 1 in, 1 out]
              n165 = Replace Array Subset(array=w402, new element=w399, index=6) -> (w401:u8[])
              n166 = Bundle By Name(cluster=w403, "Post Filter"=w401) -> (w406:T6)
            }
            frame 16 {
              n167 = Unbundle By Name(w411) -> ("Post Filter"=w410:u8[])
              n168 = Decimal String To Number(string=w413, default (0L)=u8 0 ("default (0 DBL)")) -> (number=w407:u8)  [unwired: 1 in, 1 out]
              n169 = Replace Array Subset(array=w410, new element=w407, index=7) -> (w409:u8[])
              n170 = Bundle By Name(cluster=w411, "Post Filter"=w409) -> (w414:T6)
            }
            frame 17 {
              n171 = Unbundle By Name(w419) -> ("Gain"=w418:u8[])
              n172 = Decimal String To Number(string=w421, default (0L)=u8 0 ("default (0 DBL)")) -> (number=w415:u8)  [unwired: 1 in, 1 out]
              n173 = Replace Array Subset(array=w418, new element=w415, index=0) -> (w417:u8[])
              n174 = Bundle By Name(cluster=w419, "Gain"=w417) -> (w422:T6)
            }
            frame 18 {
              n175 = Unbundle By Name(w427) -> ("Gain"=w426:u8[])
              n176 = Decimal String To Number(string=w429, default (0L)=u8 0 ("default (0 DBL)")) -> (number=w423:u8)  [unwired: 1 in, 1 out]
              n177 = Replace Array Subset(array=w426, new element=w423, index=1) -> (w425:u8[])
              n178 = Bundle By Name(cluster=w427, "Gain"=w425) -> (w430:T6)
            }
            frame 19 {
              n179 = Unbundle By Name(w435) -> ("Gain"=w434:u8[])
              n180 = Decimal String To Number(string=w437, default (0L)=u8 0 ("default (0 DBL)")) -> (number=w431:u8)  [unwired: 1 in, 1 out]
              n181 = Replace Array Subset(array=w434, new element=w431, index=2) -> (w433:u8[])
              n182 = Bundle By Name(cluster=w435, "Gain"=w433) -> (w438:T6)
            }
            frame 20 {
              n183 = Unbundle By Name(w443) -> ("Gain"=w442:u8[])
              n184 = Decimal String To Number(string=w445, default (0L)=u8 0 ("default (0 DBL)")) -> (number=w439:u8)  [unwired: 1 in, 1 out]
              n185 = Replace Array Subset(array=w442, new element=w439, index=3) -> (w441:u8[])
              n186 = Bundle By Name(cluster=w443, "Gain"=w441) -> (w446:T6)
            }
            frame 21 {
              n187 = Unbundle By Name(w451) -> ("Gain"=w450:u8[])
              n188 = Decimal String To Number(string=w453, default (0L)=u8 0 ("default (0 DBL)")) -> (number=w447:u8)  [unwired: 1 in, 1 out]
              n189 = Replace Array Subset(array=w450, new element=w447, index=4) -> (w449:u8[])
              n190 = Bundle By Name(cluster=w451, "Gain"=w449) -> (w454:T6)
            }
            frame 22 {
              n191 = Unbundle By Name(w459) -> ("Gain"=w458:u8[])
              n192 = Decimal String To Number(string=w461, default (0L)=u8 0 ("default (0 DBL)")) -> (number=w455:u8)  [unwired: 1 in, 1 out]
              n193 = Replace Array Subset(array=w458, new element=w455, index=5) -> (w457:u8[])
              n194 = Bundle By Name(cluster=w459, "Gain"=w457) -> (w462:T6)
            }
            frame 23 {
              n195 = Unbundle By Name(w467) -> ("Gain"=w466:u8[])
              n196 = Decimal String To Number(string=w469, default (0L)=u8 0 ("default (0 DBL)")) -> (number=w463:u8)  [unwired: 1 in, 1 out]
              n197 = Replace Array Subset(array=w466, new element=w463, index=6) -> (w465:u8[])
              n198 = Bundle By Name(cluster=w467, "Gain"=w465) -> (w470:T6)
            }
            frame 24 {
              n199 = Unbundle By Name(w475) -> ("Gain"=w474:u8[])
              n200 = Decimal String To Number(string=w477, default (0L)=u8 0 ("default (0 DBL)")) -> (number=w471:u8)  [unwired: 1 in, 1 out]
              n201 = Replace Array Subset(array=w474, new element=w471, index=7) -> (w473:u8[])
              n202 = Bundle By Name(cluster=w475, "Gain"=w473) -> (w478:T6)
            }
            frame 25 {
              n203 = Decimal String To Number(string=w482, default (0L)=u16 0 ("default (0 DBL)")) -> (number=w479:u16)  [unwired: 1 in, 1 out]
              n204 = Bundle By Name(cluster=w480, "FS"=w479) -> (w483:T6)
            }
            frame 26 {
              n205 = Decimal String To Number(string=w487, default (0L)=u8 0 ("default (0 DBL)")) -> (number=w484:u8)  [unwired: 1 in, 1 out]
              n206 = Bundle By Name(cluster=w485, "IntOC"=w484) -> (w488:T6)
            }
            frame 27 {
              n207 = Decimal String To Number(string=w492, default (0L)=u8 0 ("default (0 DBL)")) -> (number=w489:u8)  [unwired: 1 in, 1 out]
              n208 = Bundle By Name(cluster=w490, "IntFC"=w489) -> (w493:T6)
            }
            frame 28 {
              n209 = Decimal String To Number(string=w497, default (0L)=u8 0 ("default (0 DBL)")) -> (number=w494:u8)  [unwired: 1 in, 1 out]
              n210 = Bundle By Name(cluster=w495, "SysOC"=w494) -> (w498:T6)
            }
            frame 29 {
              n211 = Unbundle By Name(w503) -> ("Cofficient"=w502:dbl[])
              n212 = Fract/Exp String To Number(string=w505, default (0 dbl)=0.0 ("default (0 DBL)")) -> (number=w499:dbl)  [unwired: 2 in, 1 out]
              n213 = Replace Array Subset(array=w502, new element=w499, index=0) -> (w501:dbl[])
              n214 = Bundle By Name(cluster=w503, "Cofficient"=w501) -> (w506:T6)
            }
            frame 30 {
              n215 = Unbundle By Name(w511) -> ("Cofficient"=w510:dbl[])
              n216 = Fract/Exp String To Number(string=w513, default (0 dbl)=0.0 ("default (0 DBL)")) -> (number=w507:dbl)  [unwired: 2 in, 1 out]
              n217 = Replace Array Subset(array=w510, new element=w507, index=1) -> (w509:dbl[])
              n218 = Bundle By Name(cluster=w511, "Cofficient"=w509) -> (w514:T6)
            }
            frame 31 {
              n219 = Unbundle By Name(w519) -> ("Cofficient"=w518:dbl[])
              n220 = Fract/Exp String To Number(string=w521, default (0 dbl)=0.0 ("default (0 DBL)")) -> (number=w515:dbl)  [unwired: 2 in, 1 out]
              n221 = Replace Array Subset(array=w518, new element=w515, index=2) -> (w517:dbl[])
              n222 = Bundle By Name(cluster=w519, "Cofficient"=w517) -> (w522:T6)
            }
            frame 32 {
              n223 = Unbundle By Name(w527) -> ("Cofficient"=w526:dbl[])
              n224 = Fract/Exp String To Number(string=w529, default (0 dbl)=0.0 ("default (0 DBL)")) -> (number=w523:dbl)  [unwired: 2 in, 1 out]
              n225 = Replace Array Subset(array=w526, new element=w523, index=3) -> (w525:dbl[])
              n226 = Bundle By Name(cluster=w527, "Cofficient"=w525) -> (w530:T6)
            }
            frame 33 {
              n227 = Unbundle By Name(w535) -> ("Cofficient"=w534:dbl[])
              n228 = Fract/Exp String To Number(string=w537, default (0 dbl)=0.0 ("default (0 DBL)")) -> (number=w531:dbl)  [unwired: 2 in, 1 out]
              n229 = Replace Array Subset(array=w534, new element=w531, index=4) -> (w533:dbl[])
              n230 = Bundle By Name(cluster=w535, "Cofficient"=w533) -> (w538:T6)
            }
            frame 34 {
              n231 = Unbundle By Name(w543) -> ("Cofficient"=w542:dbl[])
              n232 = Fract/Exp String To Number(string=w545, default (0 dbl)=0.0 ("default (0 DBL)")) -> (number=w539:dbl)  [unwired: 2 in, 1 out]
              n233 = Replace Array Subset(array=w542, new element=w539, index=5) -> (w541:dbl[])
              n234 = Bundle By Name(cluster=w543, "Cofficient"=w541) -> (w546:T6)
            }
            frame 35 {
              n235 = Unbundle By Name(w551) -> ("Cofficient"=w550:dbl[])
              n236 = Fract/Exp String To Number(string=w553, default (0 dbl)=0.0 ("default (0 DBL)")) -> (number=w547:dbl)  [unwired: 2 in, 1 out]
              n237 = Replace Array Subset(array=w550, new element=w547, index=6) -> (w549:dbl[])
              n238 = Bundle By Name(cluster=w551, "Cofficient"=w549) -> (w554:T6)
            }
            frame 36 {
              n239 = Unbundle By Name(w559) -> ("Cofficient"=w558:dbl[])
              n240 = Fract/Exp String To Number(string=w561, default (0 dbl)=0.0 ("default (0 DBL)")) -> (number=w555:dbl)  [unwired: 2 in, 1 out]
              n241 = Replace Array Subset(array=w558, new element=w555, index=7) -> (w557:dbl[])
              n242 = Bundle By Name(cluster=w559, "Cofficient"=w557) -> (w562:T6)
            }
            frame 37 {
              n243 = Unbundle By Name(w567) -> ("K"=w566:dbl[])
              n244 = Fract/Exp String To Number(string=w569, default (0 dbl)=0.0 ("default (0 DBL)")) -> (number=w563:dbl)  [unwired: 2 in, 1 out]
              n245 = Replace Array Subset(array=w566, new element=w563, index=0) -> (w565:dbl[])
              n246 = Bundle By Name(cluster=w567, "K"=w565) -> (w570:T6)
            }
            frame 38 {
              n247 = Unbundle By Name(w575) -> ("K"=w574:dbl[])
              n248 = Fract/Exp String To Number(string=w577, default (0 dbl)=0.0 ("default (0 DBL)")) -> (number=w571:dbl)  [unwired: 2 in, 1 out]
              n249 = Replace Array Subset(array=w574, new element=w571, index=1) -> (w573:dbl[])
              n250 = Bundle By Name(cluster=w575, "K"=w573) -> (w578:T6)
            }
            frame 39 {
              n251 = Decimal String To Number(string=w582, default (0L)=0 ("Max")) -> (number=w579:i32)  [unwired: 1 in, 1 out]
              n252 = Bundle By Name(cluster=w581, "Max"=w579) -> (w583:T6)
            }
          }
        }
        n253 = Bundle By Name(cluster=T3 {"Test"={"Target Load"=0.0, "Target Disp"=0.0, "Rate"=0.0, "Speed"=0.0}, "Sensor"={"Name"=[], "Unit"=[], "Decimal Point"=[], "Ch Log"=[], "H Alarm"=[], "L Alarm"=[], "H Limit"=[], "L Limit"=[], "Filter"=[], "Gain"=[], "Calib Type"=[]}, "PID"={"SP"=0.0, "PV"=0.0, "kP"=0.0, "kI"=0.0, "kD"=0.0, "FF"=0.0, "Err Band"=0.0, "Max"=0, "Min"=0, "Ts"=0, "Out"=0, "Mode"=0}, "ADC"={"Active Ch"=[], "Filter Type"=0, "Post Filter"=[], "Gain"=[], "FS"=0, "IntOC"=0, "IntFC"=0, "SysOC"=0, "Cofficient"=[], "K"=[], "Max"=0}, "System"={"Out Type"=0, "Inverse"=0, "Monitor"=0, "Reserve"=0, "ACC Time"=0, "Pulse Rev"=0, "Stroke"=0, "Auto Off"=0, "Gear Ratio"=0.0, "Pitch"=0.0, "Max Speed"=0, "Jog Speed"=0, "Disp Coff"=0.0, "Max Load"=0}, "Index"=enum."Ch1", "Datalog"=enum."Empty"} ("Data"), "ADC"=w268) -> (w267:T3)
        n254 = call "Communication - Send Command Read.vi"("Fron?"=TRUE, "Bypass?"=TRUE, "error in (no error)"=w274, "Data"=w267, "Action"=UDP_-_Command."Write ADC", "Device IP Address"=w272) -> ("error out"=w273:errorcluster)  [unwired: 5 in]
      }
      frame "Set Sensor" {
        n255 = Index Array(array="Sensor", index (col)=1 ("disabled index (col)")) -> (element=w586:string[])  [unwired: 1 in]
        n256 = Array Size(array=w586) -> (size(s)=w589:i32)
        n257 = Subtract(x=w589, y=52) -> (x-y=w587:i32)
        n258 = case shown="..-1" w587 {
          selector: w587 -> [_ w605 w612]
          tunnel: w586 -> [w603 w607 w614]
          tunnel: [w603 w606 w613] -> w585
          frame 0, Default {
          }
          frame ..-1 {
            n259 = Absolute Value(x=w605) -> (abs(x)=w604:i32)
            n260 = for {
              N: w604 -> [_]
              tunnel: w607 -> [w610]
              tunnel: [w609] -> w606
              n261 = Insert Into Array(array=w610, new element="" ("new element/subarray")) -> (w609:string[])  [unwired: 1 in]
            }
          }
          frame 1.. {
            n262 = Absolute Value(x=w612) -> (abs(x)=w611:i32)
            n263 = Delete From Array(array=w614, length=w611) -> (array with subset deleted=w613:string[])  [unwired: 1 in, 1 out]
          }
        }
        n264 = for {
          N: 13 -> [_]
          tunnel: w585 -> [w617]
          shift-right: [w615] -> w591
          shift-left: T7 {"Name"=[], "Unit"=[], "Decimal Point"=[], "Ch Log"=[], "H Alarm"=[], "L Alarm"=[], "H Limit"=[], "L Limit"=[], "Filter"=[], "Gain"=[], "Calib Type"=[]} ("Sensor") -> [w616]
          i -> [w618]
          n265 = case shown="3" w618 {
            tunnel: w617 -> [_ w623 w627 w633 w639 w645 w651 w657 w663 w669 w675 w681 _]
            tunnel: w616 -> [w619 w622 w626 w632 w638 w644 w650 w656 w662 w668 w674 w680 w682]
            tunnel: [w619 w621 w625 w631 w637 w643 w649 w655 w661 w667 w673 w679 w682] -> w615
            frame 0, Default {
            }
            frame 1 {
              n266 = Decimate 1D Array(w623) -> (w620:string[])  [unwired: 12 out]
              n267 = Bundle By Name(cluster=w622, "Name"=w620) -> (w621:T7)
            }
            frame 2 {
              n268 = Decimate 1D Array(w627) -> (w624:string[])  [unwired: 12 out]
              n269 = Bundle By Name(cluster=w626, "Unit"=w624) -> (w625:T7)
            }
            frame 3 {
              n270 = Decimate 1D Array(w633) -> (w630:string[])  [unwired: 12 out]
              n271 = Decimal String To Number(string=w630, default (0L)=u8 0 ("default (0 I32)")) -> (number=w629:u8[])  [unwired: 1 in, 1 out]
              n272 = Bundle By Name(cluster=w632, "Decimal Point"=w629) -> (w631:T7)
            }
            frame 4 {
              n273 = Decimate 1D Array(w639) -> (w634:string[])  [unwired: 12 out]
              n274 = Decimal String To Number(string=w634, default (0L)=u8 0 ("default (0 I32)")) -> (number=w636:u8[])  [unwired: 1 in, 1 out]
              n275 = Bundle By Name(cluster=w638, "Ch Log"=w636) -> (w637:T7)
            }
            frame 5 {
              n276 = Decimate 1D Array(w645) -> (w640:string[])  [unwired: 12 out]
              n277 = Decimal String To Number(string=w640, default (0L)=u8 0 ("default (0 I32)")) -> (number=w642:u8[])  [unwired: 1 in, 1 out]
              n278 = Bundle By Name(cluster=w644, "H Alarm"=w642) -> (w643:T7)
            }
            frame 6 {
              n279 = Decimate 1D Array(w651) -> (w646:string[])  [unwired: 12 out]
              n280 = Decimal String To Number(string=w646, default (0L)=u8 0 ("default (0 I32)")) -> (number=w648:u8[])  [unwired: 1 in, 1 out]
              n281 = Bundle By Name(cluster=w650, "L Alarm"=w648) -> (w649:T7)
            }
            frame 7 {
              n282 = Decimate 1D Array(w657) -> (w652:string[])  [unwired: 12 out]
              n283 = Fract/Exp String To Number(string=w652, default (0 dbl)=sgl 0.0 ("default (0 I32)")) -> (number=w654:sgl[])  [unwired: 2 in, 1 out]
              n284 = Bundle By Name(cluster=w656, "H Limit"=w654) -> (w655:T7)
            }
            frame 8 {
              n285 = Decimate 1D Array(w663) -> (w658:string[])  [unwired: 12 out]
              n286 = Fract/Exp String To Number(string=w658, default (0 dbl)=sgl 0.0 ("default (0 I32)")) -> (number=w660:sgl[])  [unwired: 2 in, 1 out]
              n287 = Bundle By Name(cluster=w662, "L Limit"=w660) -> (w661:T7)
            }
            frame 9 {
              n288 = Decimate 1D Array(w669) -> (w665:string[])  [unwired: 12 out]
              n289 = Decimal String To Number(string=w665, default (0L)=u8 0 ("default (0 I32)")) -> (number=w666:u8[])  [unwired: 1 in, 1 out]
              n290 = Bundle By Name(cluster=w668, "Filter"=w666) -> (w667:T7)
            }
            frame 10 {
              n291 = Decimate 1D Array(w675) -> (w670:string[])  [unwired: 12 out]
              n292 = Decimal String To Number(string=w670, default (0L)=u8 0 ("default (0 I32)")) -> (number=w672:u8[])  [unwired: 1 in, 1 out]
              n293 = Bundle By Name(cluster=w674, "Gain"=w672) -> (w673:T7)
            }
            frame 11 {
              n294 = Decimate 1D Array(w681) -> (w676:string[])  [unwired: 12 out]
              n295 = Decimal String To Number(string=w676, default (0L)=u32 0 ("default (0 I32)")) -> (number=w678:u32[])  [unwired: 1 in, 1 out]
              n296 = Bundle By Name(cluster=w680, "Calib Type"=w678) -> (w679:T7)
            }
            frame 12 {
            }
          }
        }
        n297 = Bundle By Name(cluster=T3 {"Test"={"Target Load"=0.0, "Target Disp"=0.0, "Rate"=0.0, "Speed"=0.0}, "Sensor"={"Name"=[], "Unit"=[], "Decimal Point"=[], "Ch Log"=[], "H Alarm"=[], "L Alarm"=[], "H Limit"=[], "L Limit"=[], "Filter"=[], "Gain"=[], "Calib Type"=[]}, "PID"={"SP"=0.0, "PV"=0.0, "kP"=0.0, "kI"=0.0, "kD"=0.0, "FF"=0.0, "Err Band"=0.0, "Max"=0, "Min"=0, "Ts"=0, "Out"=0, "Mode"=0}, "ADC"={"Active Ch"=[], "Filter Type"=0, "Post Filter"=[], "Gain"=[], "FS"=0, "IntOC"=0, "IntFC"=0, "SysOC"=0, "Cofficient"=[], "K"=[], "Max"=0}, "System"={"Out Type"=0, "Inverse"=0, "Monitor"=0, "Reserve"=0, "ACC Time"=0, "Pulse Rev"=0, "Stroke"=0, "Auto Off"=0, "Gear Ratio"=0.0, "Pitch"=0.0, "Max Speed"=0, "Jog Speed"=0, "Disp Coff"=0.0, "Max Load"=0}, "Index"=enum."Ch1", "Datalog"=enum."Empty"} ("Data"), "Sensor"=w591) -> (w596:T3)
        n298 = call "Communication - Send Command Read.vi"("Fron?"=TRUE, "Bypass?"=TRUE, "error in (no error)"=w593, "Data"=w596, "Action"=UDP_-_Command."Write Sensor", "Device IP Address"=w594) -> ("error out"=w599:errorcluster)  [unwired: 5 in]
      }
      frame "Set PID" {
        n299 = Index Array(array="PID", index (col)=1 ("disabled index (col)")) -> (element=w689:string[])  [unwired: 1 in]
        n300 = for {
          tunnel: w689 -> [w699] mode=indexing
          shift-right: [w697] -> w687
          shift-left: T8 {"SP"=0.0, "PV"=0.0, "kP"=0.0, "kI"=0.0, "kD"=0.0, "FF"=0.0, "Err Band"=0.0, "Max"=0, "Min"=0, "Ts"=0, "Out"=0, "Mode"=0} ("PID") -> [w698]
          i -> [w700]
          n301 = case shown="10" w700 {
            tunnel: w699 -> [w703 w708 w713 w718 w723 w728 w733 w738 w743 w748 w753 w758]
            tunnel: w698 -> [w705 w710 w715 w720 w725 w730 w735 w740 w745 w750 w755 w760]
            tunnel: [w704 w709 w714 w719 w724 w729 w734 w739 w744 w749 w754 w759] -> w697
            frame 0, Default {
              n302 = Fract/Exp String To Number(string=w703, default (0 dbl)=sgl 0.0 ("default (0 DBL)")) -> (number=w702:sgl)  [unwired: 2 in, 1 out]
              n303 = Bundle By Name(cluster=w705, "SP"=w702) -> (w704:T8)
            }
            frame 1 {
              n304 = Fract/Exp String To Number(string=w708, default (0 dbl)=sgl 0.0 ("default (0 DBL)")) -> (number=w707:sgl)  [unwired: 2 in, 1 out]
              n305 = Bundle By Name(cluster=w710, "PV"=w707) -> (w709:T8)
            }
            frame 2 {
              n306 = Fract/Exp String To Number(string=w713, default (0 dbl)=sgl 0.0 ("default (0 DBL)")) -> (number=w712:sgl)  [unwired: 2 in, 1 out]
              n307 = Bundle By Name(cluster=w715, "kP"=w712) -> (w714:T8)
            }
            frame 3 {
              n308 = Fract/Exp String To Number(string=w718, default (0 dbl)=sgl 0.0 ("default (0 DBL)")) -> (number=w717:sgl)  [unwired: 2 in, 1 out]
              n309 = Bundle By Name(cluster=w720, "kI"=w717) -> (w719:T8)
            }
            frame 4 {
              n310 = Fract/Exp String To Number(string=w723, default (0 dbl)=sgl 0.0 ("default (0 DBL)")) -> (number=w722:sgl)  [unwired: 2 in, 1 out]
              n311 = Bundle By Name(cluster=w725, "kD"=w722) -> (w724:T8)
            }
            frame 5 {
              n312 = Fract/Exp String To Number(string=w728, default (0 dbl)=sgl 0.0 ("default (0 DBL)")) -> (number=w727:sgl)  [unwired: 2 in, 1 out]
              n313 = Bundle By Name(cluster=w730, "FF"=w727) -> (w729:T8)
            }
            frame 6 {
              n314 = Fract/Exp String To Number(string=w733, default (0 dbl)=sgl 0.0 ("default (0 DBL)")) -> (number=w732:sgl)  [unwired: 2 in, 1 out]
              n315 = Bundle By Name(cluster=w735, "Err Band"=w732) -> (w734:T8)
            }
            frame 7 {
              n316 = Decimal String To Number(string=w738, default (0L)=0 ("default (0 DBL)")) -> (number=w736:i32)  [unwired: 1 in, 1 out]
              n317 = Bundle By Name(cluster=w740, "Max"=w736) -> (w739:T8)
            }
            frame 8 {
              n318 = Decimal String To Number(string=w743, default (0L)=0 ("default (0 DBL)")) -> (number=w742:i32)  [unwired: 1 in, 1 out]
              n319 = Bundle By Name(cluster=w745, "Min"=w742) -> (w744:T8)
            }
            frame 9 {
              n320 = Decimal String To Number(string=w748, default (0L)=u32 0 ("Ts")) -> (number=w746:u32)  [unwired: 1 in, 1 out]
              n321 = Bundle By Name(cluster=w750, "Ts"=w746) -> (w749:T8)
            }
            frame 10 {
              n322 = Decimal String To Number(string=w753, default (0L)=0 ("Out")) -> (number=w751:i32)  [unwired: 1 in, 1 out]
              n323 = Bundle By Name(cluster=w755, "Out"=w751) -> (w754:T8)
            }
            frame 11 {
              n324 = Decimal String To Number(string=w758, default (0L)=u8 0 ("Mode")) -> (number=w756:u8)  [unwired: 1 in, 1 out]
              n325 = Bundle By Name(cluster=w760, "Mode"=w756) -> (w759:T8)
            }
          }
        }
        n326 = Bundle By Name(cluster=T3 {"Test"={"Target Load"=0.0, "Target Disp"=0.0, "Rate"=0.0, "Speed"=0.0}, "Sensor"={"Name"=[], "Unit"=[], "Decimal Point"=[], "Ch Log"=[], "H Alarm"=[], "L Alarm"=[], "H Limit"=[], "L Limit"=[], "Filter"=[], "Gain"=[], "Calib Type"=[]}, "PID"={"SP"=0.0, "PV"=0.0, "kP"=0.0, "kI"=0.0, "kD"=0.0, "FF"=0.0, "Err Band"=0.0, "Max"=0, "Min"=0, "Ts"=0, "Out"=0, "Mode"=0}, "ADC"={"Active Ch"=[], "Filter Type"=0, "Post Filter"=[], "Gain"=[], "FS"=0, "IntOC"=0, "IntFC"=0, "SysOC"=0, "Cofficient"=[], "K"=[], "Max"=0}, "System"={"Out Type"=0, "Inverse"=0, "Monitor"=0, "Reserve"=0, "ACC Time"=0, "Pulse Rev"=0, "Stroke"=0, "Auto Off"=0, "Gear Ratio"=0.0, "Pitch"=0.0, "Max Speed"=0, "Jog Speed"=0, "Disp Coff"=0.0, "Max Load"=0}, "Index"=enum."Ch1", "Datalog"=enum."Empty"} ("Data"), "PID"=w687) -> (w686:T3)
        n327 = call "Communication - Send Command Read.vi"("Fron?"=TRUE, "Bypass?"=TRUE, "error in (no error)"=w693, "Data"=w686, "Action"=UDP_-_Command."Write PID", "Device IP Address"=w691) -> ("error out"=w692:errorcluster)  [unwired: 5 in]
      }
      frame "Save" {
        w769 = T12 1 items=["User Home"=0, "User Desktop"=1, "User Documents"=2, "User Application Data"=3, "User Preferences"=4, "User Temporary"=5, "Public Documents"=6, "Public Application Data"=7, "Public Preferences"=8, "Public Cache"=13, "System Core Libraries"=9, "System Installed Libraries"=10, "Application Files"=11, "Boot Volume Root"=12] ("system directory type")
        n328 = call <vilib>:"Get System Directory.vi"("system directory type"=w769) -> ("system directory"=w768:path)  [unwired: 10 in]
        n329 = call "File Dialog"("start path"=w768, "error in"=w770, "pattern (all files)"="*.setup", "pattern label"="Machine Setting") -> ("selected path"=w763:path, "exists"=w761:bool, "cancelled"=w762:bool, "error out"=w764:errorcluster)  [unwired: 8 in]
        n330 = case shown="False" w762 {
          tunnel: [w782 w825] -> w765
          tunnel: w764 -> [w777 w826]
          tunnel: w763 -> [w778 _]
          tunnel: w761 -> [w776 _]
          frame False {
            n331 = case shown="True" w776 {
              tunnel: w777 -> [w819 w824]
              tunnel: [w819 w823] -> w780
              tunnel: w778 -> [w820 w822]
              tunnel: [w820 w821] -> w779
              frame False {
              }
              frame True {
                n332 = Delete(path (use dialog)=w822, error in=w824) -> (deleted path=w821:path, error out=w823:errorcluster)  [unwired: 3 in, 1 out]
              }
            }
            n333 = call <vilib>:"Open Config Data.vi"("error in (no error)"=w780, "configuration file path"=w779) -> ("error out"=w775:errorcluster, "refnum"=w784:T13)  [unwired: 7 in, 1 out]
            n334 = property on="Tab Control" class="TabCtl (strict)"(error in=w775) -> (error out=w774:errorcluster, "Pages"=w773:refnum<vi>[])  [unwired: 1 in, 1 out]
            n335 = for {
              shift-right: [w790] -> w783
              shift-left: w774 -> [w788]
              shift-right: [w789] -> w781
              shift-left: w784 -> [w796]
              tunnel: w773 -> [w786] mode=indexing
              n336 = property class="Page"(reference=w786, error in=w788) -> (error out=w787:errorcluster, "PageLabel"=w785:string)  [unwired: 1 out]
              n337 = case shown="\"Sensor\"" w785 {
                tunnel: [w814 w815 w816 w817 w818] -> w795
                frame "System", Default {
                  n338 = local read "System"() -> (w814:string[][])
                }
                frame "Test" {
                  n339 = local read "Test"() -> (w815:string[][])
                }
                frame "ADC" {
                  n340 = local read "ADC"() -> (w816:string[][])
                }
                frame "Sensor" {
                  n341 = local read "Sensor"() -> (w817:string[][])
                }
                frame "PID" {
                  n342 = local read "PID"() -> (w818:string[][])
                }
              }
              n343 = Index Array(array=w795, index (col) #1=0 ("disabled index (col)"), index (col) #2=1 ("index (col)")) -> (element #1=w793:string[], element #2=w791:string[])  [unwired: 2 in]
              n344 = for {
                tunnel: w785 -> [w801]
                tunnel: w793 -> [w798] mode=indexing
                shift-right: [w803] -> w790
                shift-left: w787 -> [w804]
                tunnel: w791 -> [w800] mode=indexing
                shift-right: [w799] -> w789
                shift-left: w796 -> [w802]
                n345 = Empty String/Path?(string/path=w798) -> (empty?=w797:bool)
                n346 = case shown="False" w797 {
                  tunnel: w804 -> [w805 w813]
                  tunnel: [w805 w812] -> w803
                  tunnel: w802 -> [w806 w811]
                  tunnel: w801 -> [_ w810]
                  tunnel: w800 -> [_ w809]
                  tunnel: [w806 w808] -> w799
                  tunnel: w798 -> [_ w807]
                  frame False {
                  }
                  frame True {
                    n347 = call-poly <vilib>:"Write Key.vi"("section"=w810, "error in (no error)"=w813, "value"=w809, "key"=w807, "refnum"=w811) -> ("error out"=w812:errorcluster, "refnum out"=w808:T13)  [unwired: 4 in, 1 out]
                  }
                }
              }
            }
            n348 = call <vilib>:"Close Config Data.vi"("error in (no error)"=w783, "refnum"=w781) -> ("error out"=w782:errorcluster)  [unwired: 8 in, 1 out]
          }
          frame True {
            n349 = call <vilib>:"Clear Errors.vi"("error in (no error)"=w826) -> ("error out"=w825:errorcluster)  [unwired: 5 in, 1 out]
          }
        }
      }
      frame "Load" {
        w835 = T12 1 items=["User Home"=0, "User Desktop"=1, "User Documents"=2, "User Application Data"=3, "User Preferences"=4, "User Temporary"=5, "Public Documents"=6, "Public Application Data"=7, "Public Preferences"=8, "Public Cache"=13, "System Core Libraries"=9, "System Installed Libraries"=10, "Application Files"=11, "Boot Volume Root"=12] ("system directory type")
        n350 = call <vilib>:"Get System Directory.vi"("system directory type"=w835) -> ("system directory"=w834:path)  [unwired: 10 in]
        n351 = call "File Dialog2"("start path"=w834, "error in"=w836, "pattern (all files)"="*.setup", "pattern label"="Machine Setting") -> ("selected path"=w831:path, "cancelled"=w828:bool, "error out"=w832:errorcluster)  [unwired: 8 in, 1 out]
        n352 = case shown="False" w828 {
          tunnel: w832 -> [w847 w885]
          tunnel: w831 -> [w846 _]
          tunnel: [w838 w884] -> w829
          frame False {
            n353 = call <vilib>:"Open Config Data.vi"("error in (no error)"=w847, "configuration file path"=w846) -> ("error out"=w844:errorcluster, "refnum"=w845:T13)  [unwired: 7 in, 1 out]
            n354 = call <vilib>:"Get Section Names.vi"("error in (no error)"=w844, "refnum"=w845) -> ("error out"=w841:errorcluster, "section names"=w843:string[], "refnum out"=w842:T13)  [unwired: 7 in]
            n355 = for {
              tunnel: w843 -> [w848] mode=indexing
              shift-right: [w849] -> w839
              shift-left: w842 -> [w856]
              shift-right: [w850] -> w840
              shift-left: w841 -> [w855]
              n356 = call <vilib>:"Get Key Names.vi"("section"=w848, "error in (no error)"=w855, "refnum"=w856) -> ("error out"=w853:errorcluster, "key names"=w852:string[], "refnum out"=w854:T13)  [unwired: 5 in, 1 out]
              n357 = for {
                tunnel: w852 -> [w861] mode=indexing
                tunnel: w848 -> [w860]
                shift-right: [w859] -> w849
                shift-left: w854 -> [w863]
                shift-right: [w858] -> w850
                shift-left: w853 -> [w862]
                tunnel: [w857] -> w851 mode=indexing
                n358 = call-poly <vilib>:"Read Key.vi"("section"=w860, "error in (no error)"=w862, "key"=w861, "refnum"=w863) -> ("error out"=w858:errorcluster, "value"=w857:string, "refnum out"=w859:T13)  [unwired: 4 in, 1 out]
              }
              n359 = case shown="\"Test\"" w848 {
                tunnel: w851 -> [w864 w868 w872 w876 w880]
                frame "PID" {
                  n360 = local read "PID"() -> (w867:string[][])
                  n361 = Replace Array Subset(array=w867, new element=w864, index (col)=1 ("disabled index (col)")) -> (w866:string[][])  [unwired: 1 in]
                  n362 = local write "PID"(w866) -> ()
                }
                frame "System", Default {
                  n363 = local read "System"() -> (w871:string[][])
                  n364 = Replace Array Subset(array=w871, new element=w868, index (col)=1 ("disabled index (col)")) -> (w870:string[][])  [unwired: 1 in]
                  n365 = local write "System"(w870) -> ()
                }
                frame "Test" {
                  n366 = local read "Test"() -> (w875:string[][])
                  n367 = Replace Array Subset(array=w875, new element=w872, index (col)=1 ("disabled index (col)")) -> (w874:string[][])  [unwired: 1 in]
                  n368 = local write "Test"(w874) -> ()
                }
                frame "ADC" {
                  n369 = local read "ADC"() -> (w879:string[][])
                  n370 = Replace Array Subset(array=w879, new element=w876, index (col)=1 ("disabled index (col)")) -> (w878:string[][])  [unwired: 1 in]
                  n371 = local write "ADC"(w878) -> ()
                }
                frame "Sensor" {
                  n372 = local read "Sensor"() -> (w883:string[][])
                  n373 = Replace Array Subset(array=w883, new element=w880, index (col)=1 ("disabled index (col)")) -> (w882:string[][])  [unwired: 1 in]
                  n374 = local write "Sensor"(w882) -> ()
                }
              }
            }
            n375 = call <vilib>:"Close Config Data.vi"("error in (no error)"=w840, "refnum"=w839) -> ("error out"=w838:errorcluster)  [unwired: 8 in, 1 out]
          }
          frame True {
            n376 = call <vilib>:"Clear Errors.vi"("error in (no error)"=w885) -> ("error out"=w884:errorcluster)  [unwired: 5 in, 1 out]
          }
        }
      }
      frame "Exit" {
      }
    }
  }
